vi "Perform Measurements.vi"(8 "error in":errorcluster, 9 "Measurement Context":refnum<class "Measure Call Context.lvclass">, 10 "Nominal output voltage":dbl, 11 "Reference values":T2) -> (0 "error out":errorcluster, 1 "Measurement Results":T1, 2 "Load out":refnum<k15>, 3 "Source out":refnum<k15>)   [LabVIEW 2021, in "Line Regulation_PMIC.lvlib"]
uses:
  Line Regulation_PMIC.lvlib
  Measurement Results.ctl
  <vilib>/Plug-In SDKs/Measurements/Measure Call Context/Measure Call Context.lvclass
  <vilib>/Plug-In SDKs/Measurements/Measure Call Context/Accessor/Is Canceled.vi
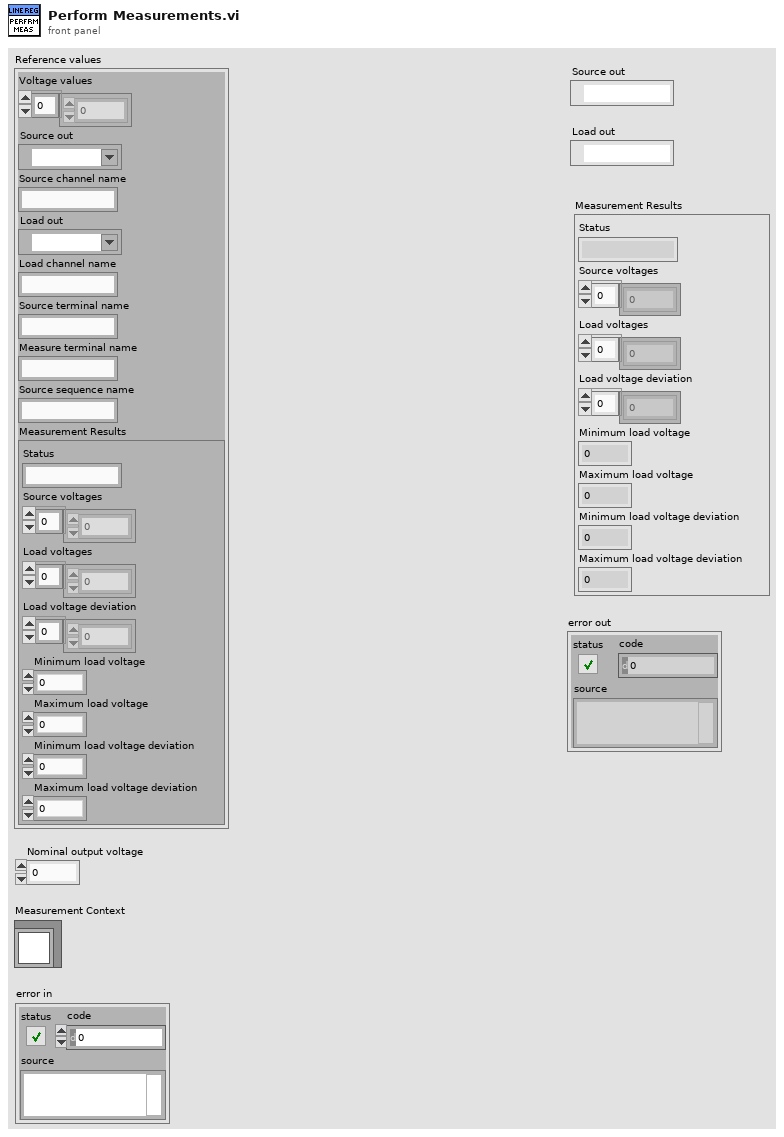
[diagram p1: front panel]
types:
  T1 = typedef "Line Regulation_PMIC.lvlib/Measurement Results.ctl" = cluster{"Status":string, "Source voltages":dbl[], "Load voltages":dbl[], "Load voltage deviation":dbl[], "Minimum load voltage":dbl, "Maximum load voltage":dbl, "Minimum load voltage deviation":dbl, "Maximum load voltage deviation":dbl}
  T2 = cluster{"Voltage values":dbl[], "Source out":refnum<k15>, "Source channel name":string, "Load out":refnum<k15>, "Load channel name":string, "Source terminal name":string, "Measure terminal name":string, "Source sequence name":string, "Measurement Results":T1}
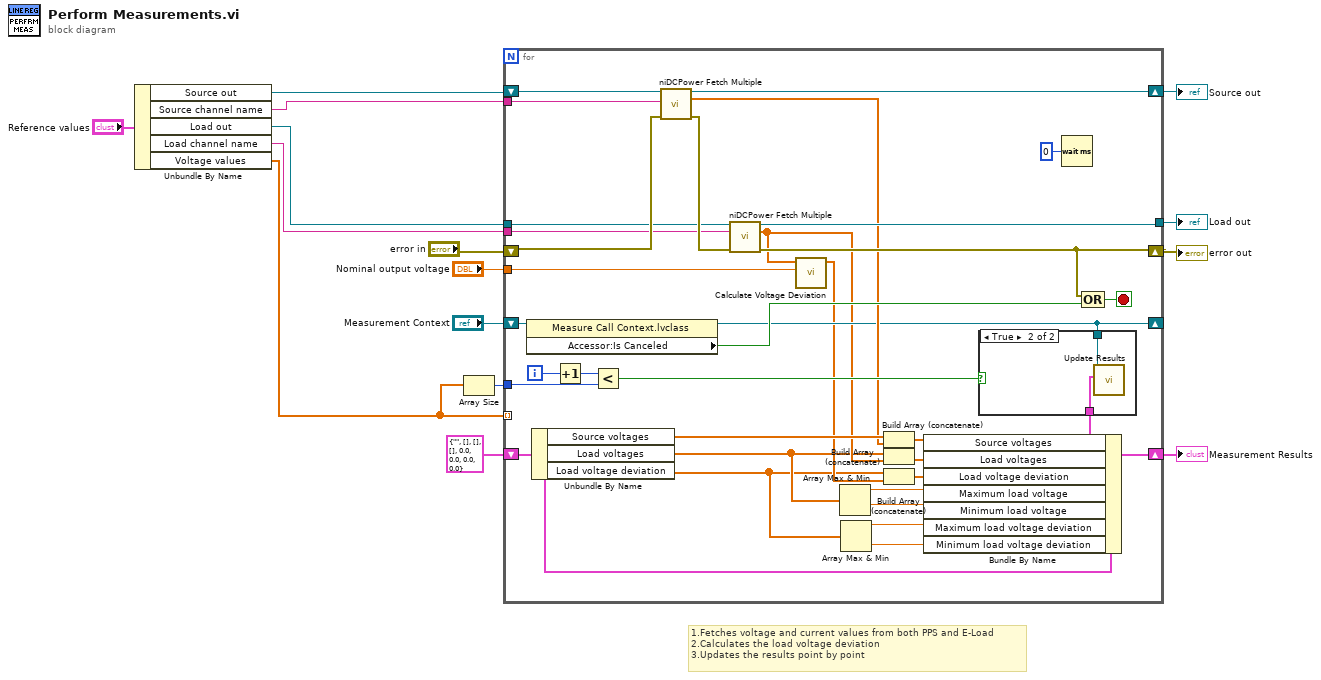
[diagram p0: block diagram]
diagram:
  # "1.Fetches voltage and current values from both PPS and E-Load\n2.Calculates the load voltage deviation\n3.Updates the results point by point"
  n1 = Unbundle By Name("Reference values") -> ("Source out"=w11:refnum<k15>, "Source channel name"=w10:string, "Load out"=w9:refnum<k15>, "Load channel name"=w8:string, "Voltage values"=w6:dbl[])
  n2 = Array Size(array=w6) -> (size(s)=w5:i32)
  n3 = for {
    shift-right: [w39] -> w14
    shift-left: "error in" -> [w45]
    shift-right: [w48] -> w4
    shift-left: w11 -> [w49]
    shift-right: [w35] -> w2
    shift-left: T1 {"Status"="", "Source voltages"=[], "Load voltages"=[], "Load voltage deviation"=[], "Minimum load voltage"=0.0, "Maximum load voltage"=0.0, "Minimum load voltage deviation"=0.0, "Maximum load voltage deviation"=0.0} ("Measurement Results") -> [w36]
    tunnel: [w47] -> w3
    shift-right: [w30] -> _
    shift-left: "Measurement Context" -> [w31]
    tunnel: w10 -> [w29]
    tunnel: w9 -> [w28]
    tunnel: w8 -> [w27]
    tunnel: "Nominal output voltage" -> [w26]
    tunnel: w6 -> [_] mode=indexing
    tunnel: w5 -> [w23]
    i -> [w44]
    stop <- w40 stop-if-true
    n4 = property class="Measure Call Context.lvclass"(reference=w31) -> (reference out=w30:refnum<class "Measure Call Context.lvclass">, "Accessor:Is Canceled"=w41:bool)  [unwired: 1 in, 1 out]
    n5 = Unbundle By Name(w36) -> ("Source voltages"=w38:dbl[], "Load voltages"=w20:dbl[], "Load voltage deviation"=w18:dbl[])
    n6 = Increment(x=w44) -> (x+1=w43:i32)
    n7 = Less?(x=w43, y=w23) -> (x < y?=w42:bool)
    n8 = call <instrlib>:"niDCPower Fetch Multiple.vi"("instrument handle"=w49, "channel name"=w29, "error in (no error)"=w45) -> ("instrument handle out"=w48:refnum<k15>, "voltage measurements"=w34:dbl[], "error out"=w46:errorcluster)  [unwired: 2 in, 8 out]
    n9 = call <instrlib>:"niDCPower Fetch Multiple.vi"("instrument handle"=w28, "channel name"=w27, "error in (no error)"=w46) -> ("instrument handle out"=w47:refnum<k15>, "voltage measurements"=w25:dbl[], "error out"=w39:errorcluster)  [unwired: 2 in, 8 out]
    n10 = call "Calculate Voltage Deviation.vi"("Nominal output voltage"=w26, "Voltage measurements"=w25) -> ("Load voltage deviation"=w24:dbl[])  [unwired: 9 in]
    n11 = Array Max & Min(array=w20) -> (max value=w19:dbl, min value=w21:dbl)  [unwired: 2 out]
    n12 = Array Max & Min(array=w18) -> (max value=w17:dbl, min value=w16:dbl)  [unwired: 2 out]
    n13 = Build Array (concatenate)(w38, w34) -> (w37:dbl[])
    n14 = Build Array (concatenate)(w20, w25) -> (w33:dbl[])
    n15 = Build Array (concatenate)(w18, w24) -> (w32:dbl[])
    n16 = Bundle By Name(cluster=w36, "Source voltages"=w37, "Load voltages"=w33, "Load voltage deviation"=w32, "Maximum load voltage"=w19, "Minimum load voltage"=w21, "Maximum load voltage deviation"=w17, "Minimum load voltage deviation"=w16) -> (w35:T1)
    n17 = case shown="True" w42 {
      tunnel: w30 -> [_ w51]
      tunnel: w35 -> [_ w50]
      frame False {
      }
      frame True {
        n18 = call <vilib>:"Update Results.vi"("measurement results"=w50, "measure call context in"=w51) -> ()  [unwired: 8 in, 2 out]
      }
    }
    n19 = Wait (ms)(milliseconds to wait=u32 0) -> ()  [unwired: 1 out]
    n20 = Compound Arithmetic op=OR(w39, w41) -> (w40:bool)
  }
  "error out" <- w14
  "Source out" <- w4
  "Load out" <- w3
  "Measurement Results" <- w2
